vi "Mise en forme graphe EPC.vi"(0 "Début du profil":timestamp format="%<%H:%M:%S\n%A %d/%m/%y>T", 1 "Port COM run 1 REG":refnum<visa-resource-name> caption="Port RS232", 2 "Val T ini en entrée":dbl, 3 "Onglet_Tinit":enum32{"Définir Tinit", "Acquérir Tinit"}(tab), 4 "Config + programmes":T2 {"Prog 10 en sortie"."?" format="%.2f"; "Prog 9 en sortie"."?" format="%.2f"; "Prog 8 en sortie"."?" format="%.2f"; "Prog 7 en sortie"."?" format="%.2f"; "Prog 6 en sortie"."?" format="%.2f"; "Prog 5 en sortie"."?" format="%.2f"; "config"."value" format="%.2f"; "Prog 1 en sortie"."?" format="%.2f"; "Prog 2 en sortie"."?" format="%.2f"; "Prog 3 en sortie"."?" format="%.2f"; "Prog 4 en sortie"."?" format="%.2f"}, 5 "adresse reg":u8) -> (6 "Graphe XY":cluster{"Y":dbl[], "Y":dbl[]}[](array[cluster]), 8 "Courbes à afficher":bool[](array[boolean]), 9 "Bornes profil":T1)   [LabVIEW 2022 SP3]
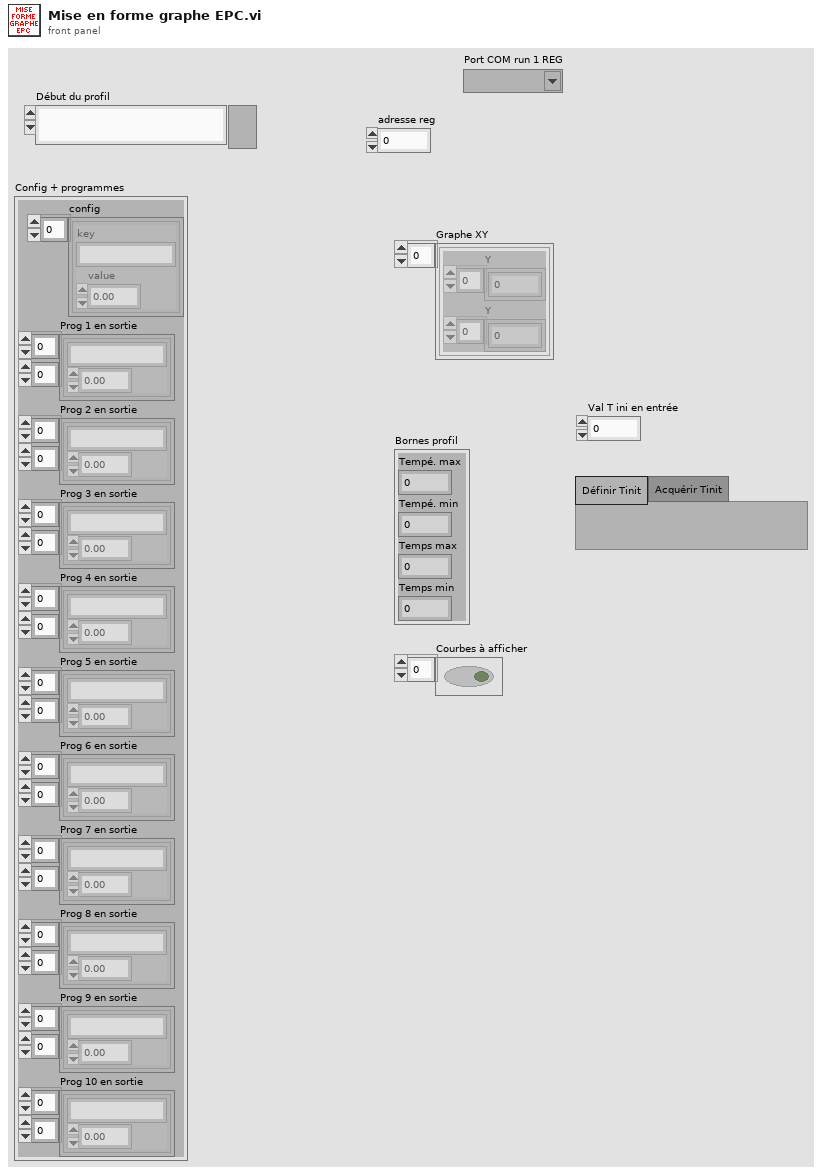
[diagram p1: front panel]
types:
  T1 = cluster{"Tempé. max":dbl, "Tempé. min":dbl, "Temps max":dbl, "Temps min":dbl}
  T2 = cluster{"config":cluster{"key":string, "value":dbl}[], "Prog 1 en sortie":cluster{string, dbl}[][], "Prog 2 en sortie":cluster{string, dbl}[][], "Prog 3 en sortie":cluster{string, dbl}[][], "Prog 4 en sortie":cluster{string, dbl}[][], "Prog 5 en sortie":cluster{string, dbl}[][], "Prog 6 en sortie":cluster{string, dbl}[][], "Prog 7 en sortie":cluster{string, dbl}[][], "Prog 8 en sortie":cluster{string, dbl}[][], "Prog 9 en sortie":cluster{string, dbl}[][], "Prog 10 en sortie":cluster{string, dbl}[][]}
  T3 = cluster{"Ev_Saut":dbl[], "Ev_Palier":dbl[], "Ev_Rampe_vitesse":dbl[], "Ev_Rampe_temps":dbl[], "Ev_Appel":dbl[], "Ev_Fin":dbl[], "T_Fin":dbl[], "T_Appel":dbl[], "T_Rampe_temps":dbl[], "T_Rampe_vitesse":dbl[], "T_Palier":dbl[], "T_Saut":dbl[], "Type de fin":string}
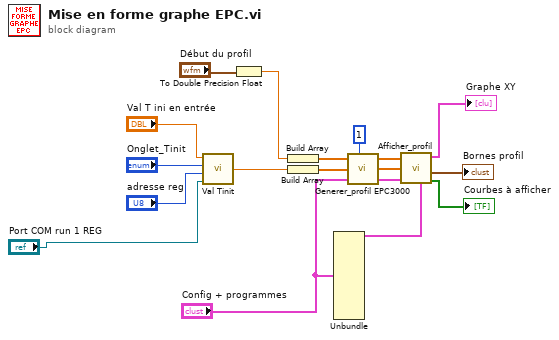
[diagram p0: block diagram]
diagram:
  n1 = call "Val Tinit.vi"("Port COM run 1 REG"="Port COM run 1 REG", "Adresse"="adresse reg", "Onglet_Tinit"="Onglet_Tinit", "Val T ini"="Val T ini en entrée") -> ("Température"=w16:dbl)
  n2 = To Double Precision Float(number="Début du profil") -> (double precision float=w13:dbl)
  n3 = Build Array(w13) -> (w6:dbl[])
  n4 = Build Array(w16) -> (w5:dbl[])
  n5 = Unbundle("Config + programmes") -> ("config"=w12:cluster{"key":string, "value":dbl}[])  [unwired: 10 out]
  n6 = call "Generer_profil EPC3000.vi"("Temps (s)"=w6, "Num_Prog"=u8 1, "Températures (°C)"=w5, "Programmes et config"="Config + programmes") -> ("Temps (s)"=w7:dbl[], "Températures (°C)"=w9:dbl[], "Evennements_sortie"=w8:T3)  [unwired: 1 in]
  n7 = call "Afficher_profil.vi"("Configuration"=w12, "Temps (s)"=w7, "Températures (°C)"=w9, "Evennements_entrée"=w8) -> ("Graphe XY"=→"Graphe XY":cluster{"Y":dbl[], "Y":dbl[]}[], "Bornes profil"=→"Bornes profil":T1, "Courbes à afficher"=→"Courbes à afficher":bool[])  [unwired: 1 out]
